vi "Wire in Main Measurement.vi"(11 "error in":errorcluster) -> (15 "error out":errorcluster)   [LabVIEW 2021, in "Migrator.lvlib"]
uses:
  Migrator.lvlib
  Path Functions/Path Functions.lvlib
  <vilib>/Utility/traverseref.llb/VI Scripting - Traverse.lvlib
  <vilib>/Utility/traverseref.llb/TRef TravTarget.ctl
  Reusables/Reusables.lvlib
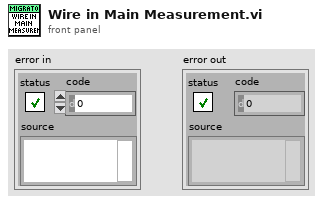
[diagram p1: front panel]
types:
  T1 = typedef "TRef TravTarget.ctl" = enum16{"FP", "BD", "Other"}
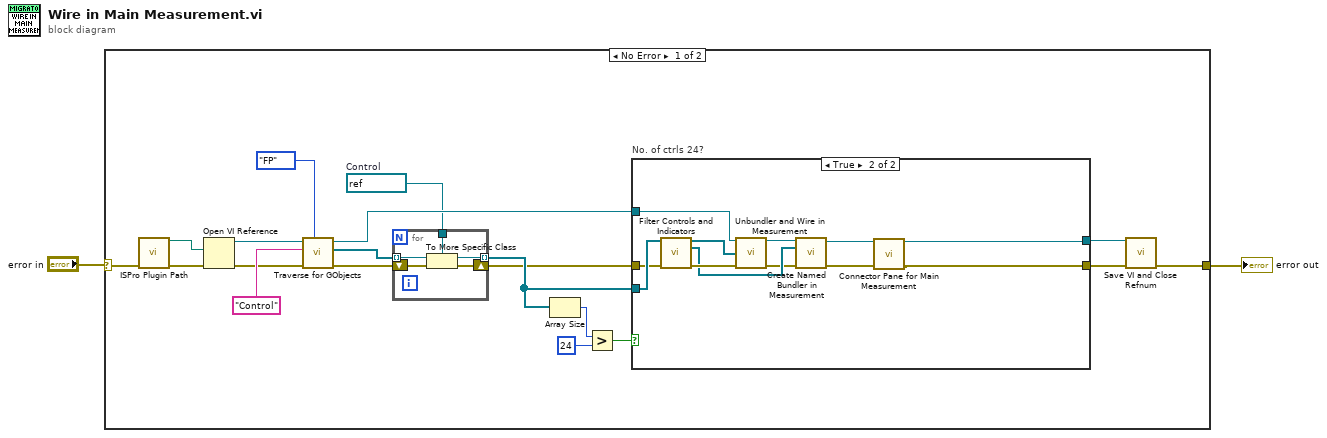
[diagram p0: block diagram]
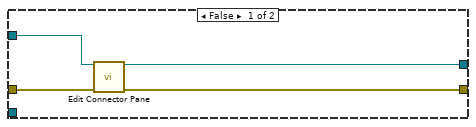
[diagram p2: hidden frame]
diagram:
  n1 = case shown="No Error" "error in" {
    selector: "error in" -> [w18 w43]
    tunnel: [w4 w43] -> w1
    frame No Error {
      w6 = refnum<vi> refnum  # Control
      n2 = call "ISPro Plugin Path.vi"("error in (no error)"=w18) -> ("Main Measurement"=w20:path, "error out"=w21:errorcluster)  [unwired: 2 in, 11 out]
      n3 = Open VI Reference(vi path=w20, error in (no error)=w21) -> (vi reference=w11:refnum<vi>, error out=w9:errorcluster)  [unwired: 4 in]
      n4 = call <vilib>:"Traverse for GObjects.vi"("Traverse Target"=TRef_TravTarget."FP", "error in (no error)"=w9, "Class Name"="Control", "VI Refnum"=w11) -> ("error out"=w8:errorcluster, "References"=w13:refnum<vi>[], "dup VI Refnum"=w10:refnum<vi>)  [unwired: 4 in, 1 out]
      n5 = for {
        tunnel: w13 -> [w26] mode=indexing
        tunnel: [w25] -> w12 mode=indexing
        shift-right: [w23] -> w7
        shift-left: w8 -> [w24]
        tunnel: w6 -> [w22]
        n6 = To More Specific Class(target class=w22, reference=w26, error in=w24) -> (specific class reference=w25:refnum<vi>, error out=w23:errorcluster)
      }
      n7 = Array Size(array=w12) -> (size(s)=w19:i32)
      n8 = Greater?(x=w19, y=24) -> (0:w16:bool)
      n9 = case "No. of ctrls 24?" shown="True" w16 {
        tunnel: w7 -> [w28 w39]
        tunnel: w10 -> [w30 w38]
        tunnel: w12 -> [_ w42]
        tunnel: [w27 w32] -> w3
        tunnel: [w29 w33] -> w5
        frame False {
          n10 = call "Edit Connector Pane.vi"("Measurement VI"=w30, "error in (no error)"=w28) -> ("Measurement VI Out"=w29:refnum<vi>, "error out"=w27:errorcluster)  [unwired: 12 in]
        }
        frame True {
          n11 = call "Filter Controls and Indicators.vi"("Controls[]"=w42, "error in (no error)"=w39) -> ("Controls[]"=w40:refnum<vi>[], "Indicators[]"=w37:refnum<vi>[], "error out"=w41:errorcluster)  [unwired: 11 in]
          n12 = call "Unbundler and Wire in Measurement.vi"("VI in"=w38, "Controls[]"=w40, "error in (no error)"=w41) -> ("VI Out"=w35:refnum<vi>, "error out"=w36:errorcluster)  [unwired: 11 in]
          n13 = call "Create Named Bundler in Measurement.vi"("VI in"=w35, "Indicators[]"=w37, "error in (no error)"=w36) -> ("VI out"=w34:refnum<vi>, "error out"=w31:errorcluster)  [unwired: 11 in]
          n14 = call "Connector Pane for Main Measurement.vi"("VI in"=w34, "error in"=w31) -> ("VI out"=w33:refnum<vi>, "error out"=w32:errorcluster)  [unwired: 12 in]
        }
      }
      n15 = call "Save VI and Close Refnum.vi"("VI Refnum"=w5, "error in"=w3) -> ("error out"=w4:errorcluster)  [unwired: 13 in]
    }
    frame Error {
    }
  }
  "error out" <- w1
